vi "ErrorSubPanelVIMissing.vi"(0 "Create Error?":bool, 5 "VI Name":string, 11 "error in":errorcluster) -> (15 "error out":errorcluster)   [LabVIEW 2016, in "Drona.lvlib"]
doc: "Creates error if the VI is not found in the SubPanel"
uses:
  Drona.lvlib
  <vilib>/Utility/error.llb/Error Cluster From Error Code.vi
  <vilib>/ErrorRing/Error Ring.xnode
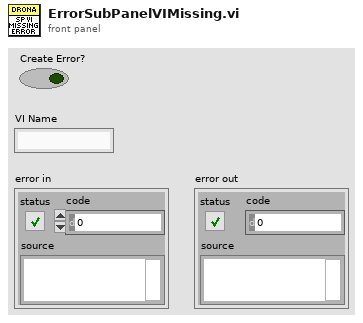
[diagram p1: front panel]
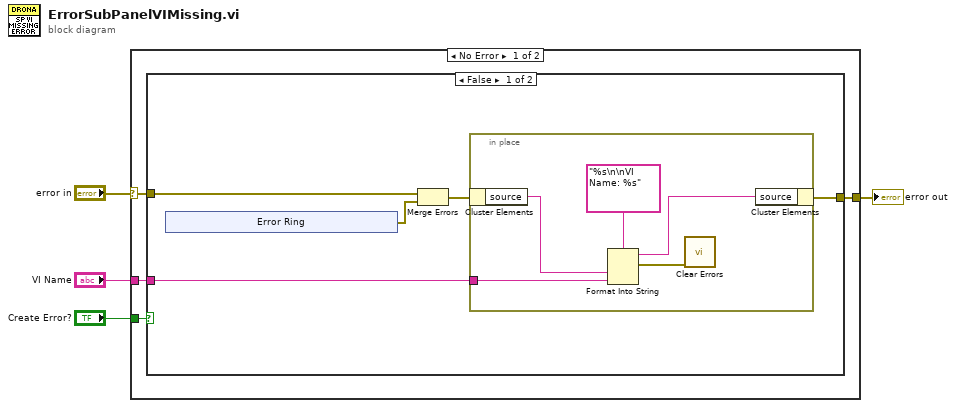
[diagram p0: block diagram]
diagram:
  n1 = case shown="No Error" "error in" {
    selector: "error in" -> [w5 w25]
    tunnel: "VI Name" -> [w8 _]
    tunnel: [w7 w25] -> w3
    tunnel: "Create Error?" -> [w6 _]
    frame No Error {
      n2 = case shown="False" w6 {
        tunnel: w5 -> [w13 w24]
        tunnel: [w11 w24] -> w7
        tunnel: w8 -> [w10 _]
        frame False {
          n3 = xnode "Error Ring"() -> ("error out"=w9:errorcluster)
          n4 = Merge Errors(w13, w9) -> (w12:errorcluster)
          n5 = in-place {
            in-place-border: w10 -> [w23]
            n6 = in-place-cluster #1(w12) -> ("source"=w20:string)
            n7 = Format Into String(format string="%s\n\nVI Name: %s", w20, w23) -> (resulting string=w21:string, error out=w19:errorcluster)  [unwired: 2 in]
            n8 = call <vilib>:"Clear Errors.vi"("error in (no error)"=w19) -> ()  [unwired: 5 in, 2 out]
            n9 = in-place-cluster #1("source"=w21) -> (w11:errorcluster)
          }
        }
        frame True {
        }
      }
    }
    frame Error {
    }
  }
  "error out" <- w3
